vi "UE_Load_Fraction.vi"(1 "fraction":dbl, 2 "reference_load_N":dbl) -> (0 "commanded_load_N":dbl)   [LabVIEW 2026]
doc: "INTENT: Calculate a configured fraction of previously measured reference load. INPUTS: reference_load_N (double), fraction (double). OUTPUTS: commanded_load_N (double). DESIGN CONSTRAINT: Used for maintenance-of-lift planning; validated fraction expected in [0,1]. REQUIREMENTS: SRS-F-008. No physical hardware side effects. Acceptance requires native LabVIEW compilation and behavioral testing."
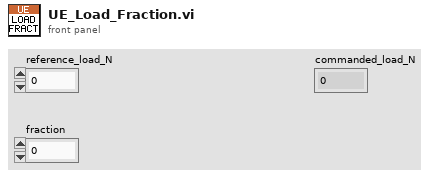
[diagram p1: front panel]
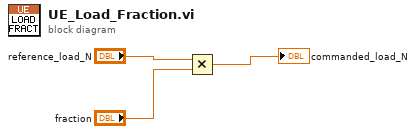
[diagram p0: block diagram]
diagram:
  n1 = Multiply(x="reference_load_N", y="fraction") -> (x*y=→"commanded_load_N":dbl)
